vi "Add Device Properties.vi"(8 "error in (no error)":errorcluster, 11 "Modbus in":refnum<class "Modbus.lvclass">) -> (0 "error out":errorcluster, 3 "Modbus out":refnum<class "Modbus.lvclass">)   [LabVIEW 2026, in "Modbus.lvlib" / "Modbus.lvclass"]
uses:
  Modbus.lvclass
  Types/Order.ctl
  Utility/Signed Representation/Types/Signed Representation.ctl
  4a14e9f2-04af-4a1e-b6b4-48975bbb3021.vi
  c6a138cd-bede-49ac-adbc-c611617db707.vi
  4a14e9f2-04af-4a1e-b6b4-48975bbb3021.vi/407e0540-03f6-4363-afc5-a4b1f046ef19.vi
  4a14e9f2-04af-4a1e-b6b4-48975bbb3021.vi/520d475a-7b95-4b20-931b-ccc2be82a762.vi
  c6a138cd-bede-49ac-adbc-c611617db707.vi/407e0540-03f6-4363-afc5-a4b1f046ef19.vi
  c6a138cd-bede-49ac-adbc-c611617db707.vi/520d475a-7b95-4b20-931b-ccc2be82a762.vi
  Globals/Modbus Strings.vi
  <vilib>/FlexLogger/SDK/PluginSDK.lvlibp/PEFClasses/SDK/Plugin/ParameterAccess/Write I32.vi
  <vilib>/FlexLogger/SDK/PluginSDK.lvlibp/PEFClasses/SDK/Plugin/ParameterAccess/Write Enum.vi
  <vilib>/FlexLogger/SDK/PluginSDK.lvlibp/PEFClasses/SDK/Plugin/Plugin.lvclass
  Utility/Utility.lvlib
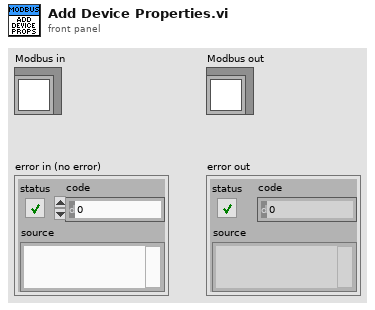
[diagram p1: front panel]
types:
  T1 = typedef "Utility.lvlib/Signed Representation.ctl" = enum16{"Two's Complement", "Offset Binary", "Sign-Magnitude", "Ones' Complement"}
  T2 = typedef "Modbus.lvlib/Modbus.lvclass/Order.ctl" = enum16{"Big-Endian (AB CD)", "Word-Swap (CD AB)", "Byte-Swap (BA DC)", "Little-Endian (DC BA)"}
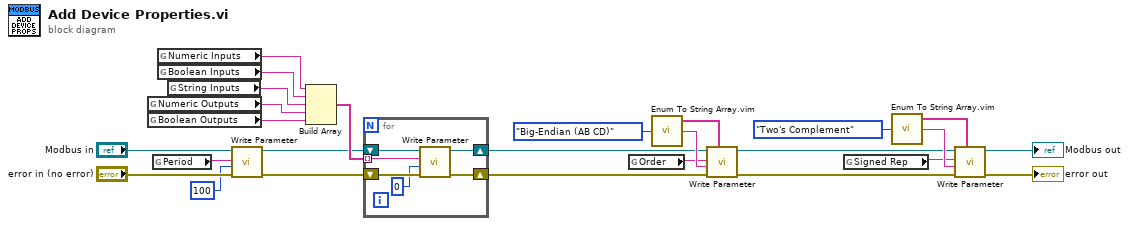
[diagram p0: block diagram]
diagram:
  n1 = global read "Modbus Strings.vi" "Numeric Outputs"() -> (w20:string)
  n2 = global read "Modbus Strings.vi" "Boolean Outputs"() -> (w19:string)
  n3 = global read "Modbus Strings.vi" "Period"() -> (w1:string)
  n4 = global read "Modbus Strings.vi" "Numeric Inputs"() -> (w18:string)
  n5 = global read "Modbus Strings.vi" "Boolean Inputs"() -> (w22:string)
  n6 = global read "Modbus Strings.vi" "String Inputs"() -> (w21:string)
  n7 = call-poly <vilib>:"Write Parameter.vi"("error in (no error)"="error in (no error)", "Value"=100, "Name"=w1, "Plugin in"="Modbus in") -> ("error out"=w3:errorcluster, "Plugin out"=w4:refnum<class "Modbus.lvclass">)  [unwired: 6 in]
  n8 = Build Array(w18, w22, w21, w20, w19) -> (w23:string[])
  n9 = for {
    shift-right: [w31] -> w5
    shift-left: w4 -> [w32]
    shift-right: [w29] -> w6
    shift-left: w3 -> [w30]
    tunnel: w23 -> [w27] mode=indexing
    n10 = call-poly <vilib>:"Write Parameter.vi"("error in (no error)"=w30, "Value"=0, "Name"=w27, "Plugin in"=w32) -> ("error out"=w29:errorcluster, "Plugin out"=w31:refnum<class "Modbus.lvclass">)  [unwired: 6 in]
  }
  n11 = global read "Modbus Strings.vi" "Order"() -> (w8:string)
  n12 = call "Enum To String Array.vim"("Enum in"=Order."Big-Endian (AB CD)" ("Order")) -> ("Selected String out"=w16:string, "Strings out"=w13:string[])  [unwired: 2 in, 1 out]
  n13 = call-poly <vilib>:"Write Parameter.vi"("Possible Values"=w13, "error in (no error)"=w6, "Current Value"=w16, "Name"=w8, "Plugin in"=w5) -> ("error out"=w11:errorcluster, "Plugin out"=w10:refnum<class "Modbus.lvclass">)  [unwired: 5 in]
  n14 = global read "Modbus Strings.vi" "Signed Rep"() -> (w9:string)
  n15 = call "Enum To String Array.vim"("Enum in"=Signed_Representation."Two's Complement" ("Signed Representation")) -> ("Selected String out"=w17:string, "Strings out"=w15:string[])  [unwired: 2 in, 1 out]
  n16 = call-poly <vilib>:"Write Parameter.vi"("Possible Values"=w15, "error in (no error)"=w11, "Current Value"=w17, "Name"=w9, "Plugin in"=w10) -> ("error out"=→"error out":errorcluster, "Plugin out"=→"Modbus out":refnum<class "Modbus.lvclass">)  [unwired: 5 in]
